vi "PathPlanner_Trajectory_WriteCSVFile.vi"(9 "Comment":string, 10 "TRAJECTORY":T1 {"States"."TargetHolonomicRotation"."SIN" format="%13.4f"; "States"."TargetHolonomicRotation"."COS" format="%13.4f"; "States"."TargetHolonomicRotation"."VALUE" format="%13.4f"; "States"."Heading"."SIN" format="%13.4f"; "States"."Heading"."COS" format="%13.4f"; "States"."Heading"."VALUE" format="%13.4f"; "States"."PositionMeters"."Y" format="%14.3f"; "States"."PositionMeters"."X" format="%14.3f"}, 11 "FileName":string="trajectory.csv") -> (0 "error out":errorcluster)   [LabVIEW 2019, in "PathPlanner24.lvlib"]
doc: "Create a CSV file from a trajectory. This can be used on a PC or the RoboRIO. \n\nParameters:\n - FileName -- Name of the CSV file to read. See file name notes for additional information.\n - Trajectory - Trajectory data structure cluster\n - Comment - string - Optional comment to place in CSV file.\n\nReturns:\n - Error out - returned error cluster\n\nNotes on file naming:\n -- The file name must include the extention. \".csv\" is not automatically appended to the name. \n -- The file name can be a simple file or an absolute path. If a simple file name is used the default path on the RoboRIO is: \"home:\\lvuser\\natinst\\LabVIEW Data\". On a Windows PC the default path is the LabVIEW default directory. Normally this is: “%HOMEDRIVE%%HOMEPATH%\\Documents\\LabView Data\".\n -- Filenames on the RoboRIO, which runs Linux, are case sensitive.\n\nNotes on file contents:\n -- Blank lines are ignored.\n -- Lines that begin with either #, !, or ' in the first character are considered comments and are ignored. \n -- Other lines are interpretted as comma separated data"
uses:
  PathPlanner24.lvlib
  TypeDef/PathPlannerTrajectory.ctl
  TypeDef/PathPlannerTrajectoryState.ctl
  <vilib>/Rock Robotics/WPI/ThirdParty/JAS_Junk/TrajLib/TypeDef/TRANSLATION2D.ctl
  <vilib>/Rock Robotics/WPI/ThirdParty/JAS_Junk/TrajLib/TypeDef/ROTATION2D.ctl
  TypeDef/PathPlannerPathConstraints.ctl
  <vilib>/Rock Robotics/WPI/ThirdParty/JAS_Junk/TrajLib/Trajectory_Library.lvlib
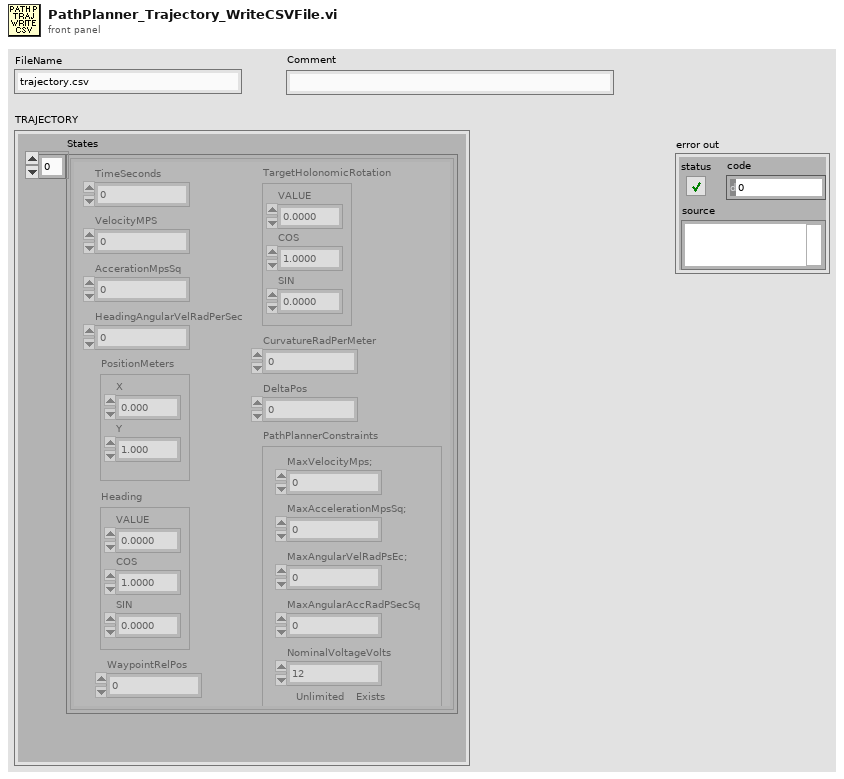
[diagram p1: front panel]
types:
  T1 = typedef "PathPlanner24.lvlib/PathPlannerTrajectory.ctl" = cluster{"States":T2[]}
  T2 = typedef "PathPlanner24.lvlib/PathPlannerTrajectoryState.ctl" = cluster{"TimeSeconds":dbl, "VelocityMPS":dbl, "AccerationMpsSq":dbl, "HeadingAngularVelRadPerSec":dbl, "PositionMeters":T3, "Heading":T4, "TargetHolonomicRotation":T4, "CurvatureRadPerMeter":dbl, "PathPlannerConstraints":T5, "DeltaPos":dbl, "WaypointRelPos":dbl}
  T3 = typedef "Trajectory_Library.lvlib/TRANSLATION2D.ctl" = cluster{"X":dbl, "Y":dbl}
  T4 = typedef "Trajectory_Library.lvlib/ROTATION2D.ctl" = cluster{"VALUE":dbl, "COS":dbl, "SIN":dbl}
  T5 = typedef "PathPlanner24.lvlib/PathPlannerPathConstraints.ctl" = cluster{"MaxVelocityMps;":dbl, "MaxAccelerationMpsSq;":dbl, "MaxAngularVelRadPsEc;":dbl, "MaxAngularAccRadPSecSq":dbl, "Exists":bool, "Unlimited":bool, "NominalVoltageVolts":dbl}
  T6 = enum16{"open", "replace", "create", "open or create", "replace or create", "replace or create with confirmation"}
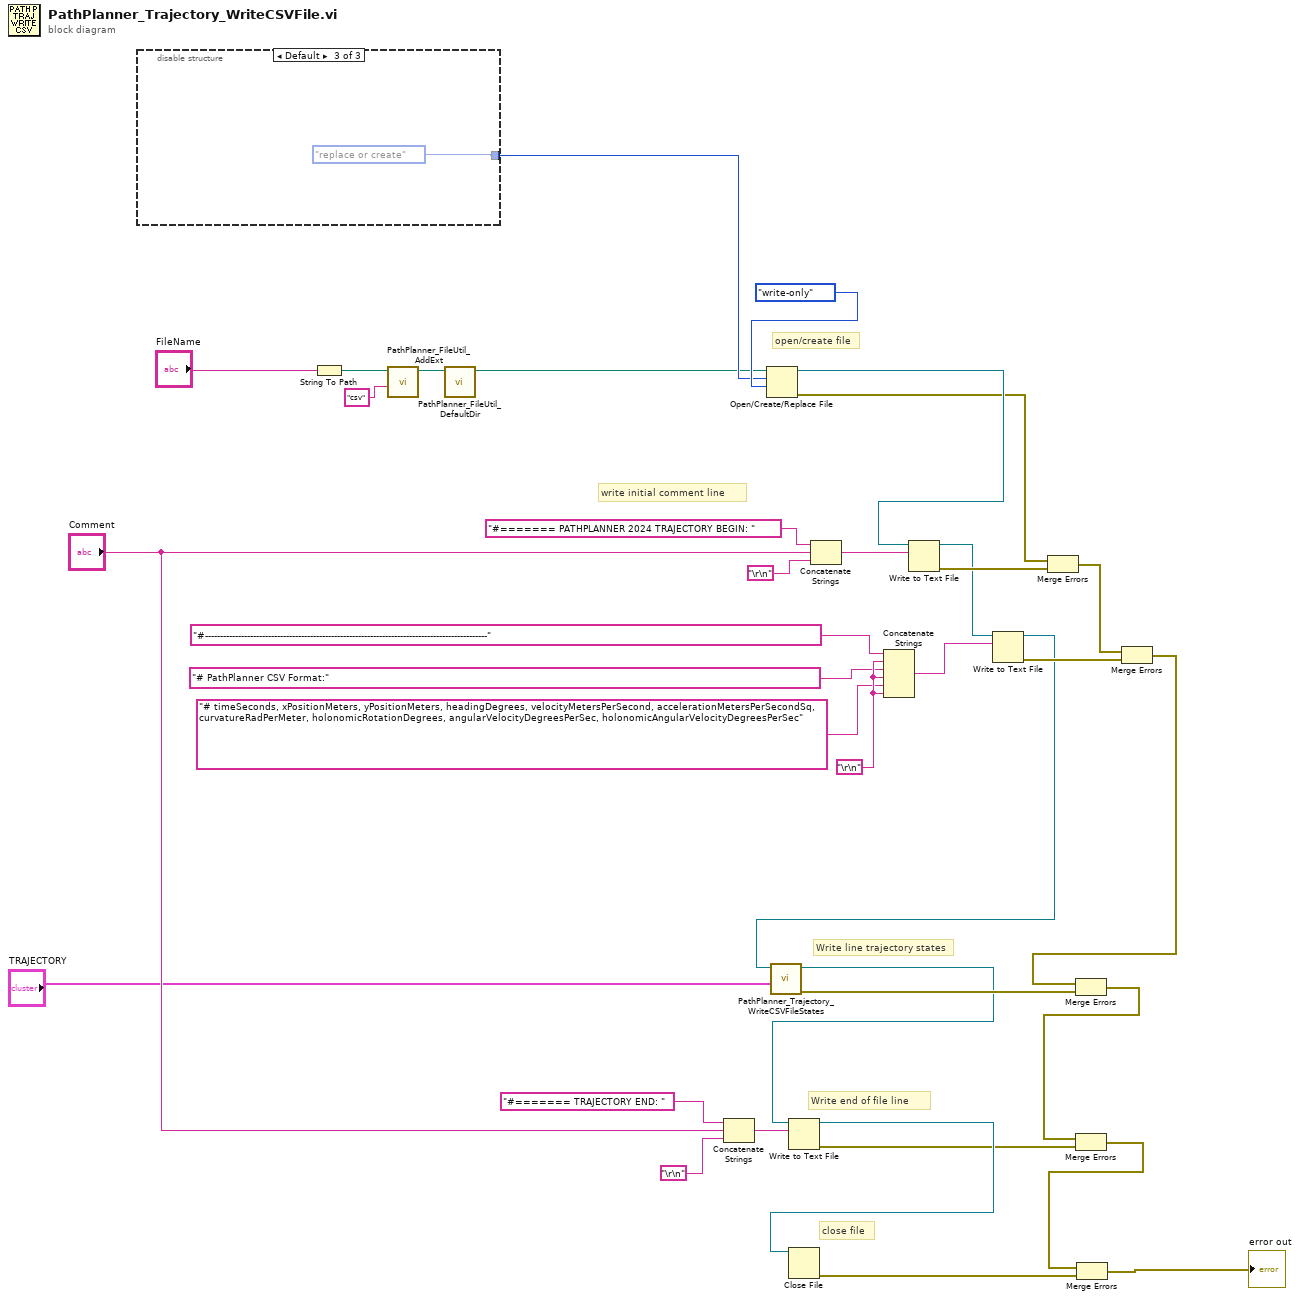
[diagram p0: block diagram]
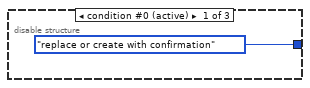
[diagram p2: hidden frame]
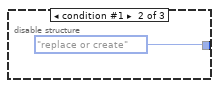
[diagram p3: hidden frame]
diagram:
  w7 = "\r\n"
  # "Write line trajectory states"
  # "open/create file"
  # "close file"
  # "Write end of file line"
  # "write initial comment line"
  n1 = disable-structure shown="Default" {
    disable-tunnel: [T6."replace or create with confirmation" ("operation (0:open)") T6."replace or create" ("operation (0:open)") T6."replace or create" ("operation (0:open)")] -> w16
    frame condition #0 (active) {
    }
    frame condition #1 {
    }
    frame condition #2 {
    }
  }
  n2 = String To Path(string="FileName") -> (path=w2:path)
  n3 = call "PathPlanner_FileUtil_AddExt.vi"("Extension"="csv", "Path in"=w2) -> ("Path out"=w4:path)  [unwired: 9 in]
  n4 = call "PathPlanner_FileUtil_DefaultDir.vi"("Path in"=w4) -> ("Path Out"=w1:path)  [unwired: 10 in]
  n5 = Concatenate Strings("#======= TRAJECTORY END: " ("string"), "Comment", "\r\n") -> (w30:string)
  n6 = Open/Create/Replace File(file path (use dialog)=w1, operation (0:open)=w16, access (0:read/write)=enum16{"read/write", "read-only", "write-only"}."write-only") -> (refnum out=w28:refnum<file>, error out=w24:errorcluster)  [unwired: 3 in, 1 out]
  n7 = Concatenate Strings("#======= PATHPLANNER 2024 TRAJECTORY BEGIN: " ("string"), "Comment", "\r\n") -> (w34:string)
  n8 = Concatenate Strings("#----------------------------------------------------------------------------------------------" ("string"), w7, "# PathPlanner CSV Format:" ("string"), w7, "# timeSeconds, xPositionMeters, yPositionMeters, headingDegrees, velocityMetersPerSecond, accelerationMetersPerSecondSq, curvatureRadPerMeter, holonomicRotationDegrees, angularVelocityDegreesPerSec, holonomicAngularVelocityDegreesPerSec" ("string"), w7) -> (w18:string)
  n9 = Write to Text File(file (use dialog)=w28, text=w34) -> (refnum out=w14:refnum<file>, error out=w25:errorcluster)  [unwired: 2 in, 1 out]
  n10 = Write to Text File(file (use dialog)=w14, text=w18) -> (refnum out=w10:refnum<file>, error out=w17:errorcluster)  [unwired: 2 in, 1 out]
  n11 = call "PathPlanner_Trajectory_WriteCSVFileStates.vi"("Trajectory"="TRAJECTORY", "Byte Steam File In"=w10) -> ("error out"=w12:errorcluster, "Byte Steam File Out"=w11:refnum<file>)  [unwired: 8 in]
  n12 = Write to Text File(file (use dialog)=w11, text=w30) -> (refnum out=w26:refnum<file>, error out=w22:errorcluster)  [unwired: 2 in, 1 out]
  n13 = Close File(refnum=w26) -> (error out=w21:errorcluster)  [unwired: 1 in, 1 out]
  n14 = Merge Errors(w24, w25) -> (w15:errorcluster)
  n15 = Merge Errors(w15, w17) -> (w13:errorcluster)
  n16 = Merge Errors(w13, w12) -> (w23:errorcluster)
  n17 = Merge Errors(w23, w22) -> (w20:errorcluster)
  n18 = Merge Errors(w20, w21) -> (→"error out":errorcluster)
